vi "OwnMergePanelInventory.vi"() -> ()   [LabVIEW 2024]
panel:
  out "error out":errorcluster caption="错误输出"
  out "pane_ids":refnum<vi>[](array[refnum])
  out "decoration_ids":refnum<vi>[](array[refnum])
  out "all_object_ids":refnum<vi>[](array[refnum])
  in  "target_path":path
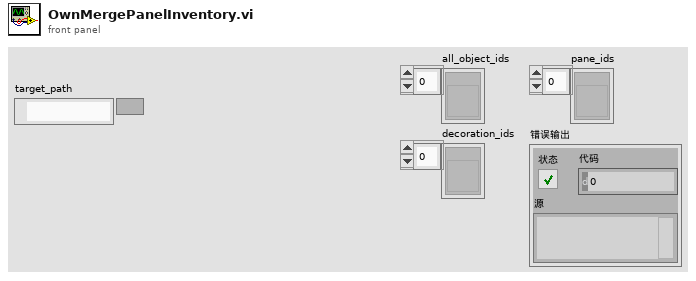
[diagram p1: front panel]
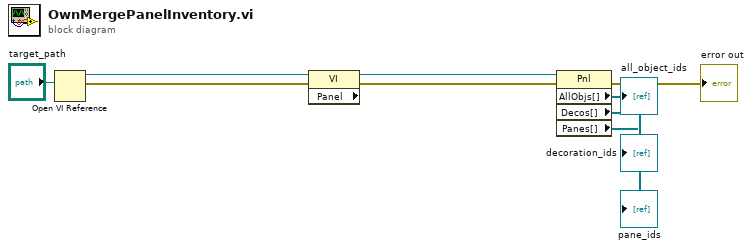
[diagram p0: block diagram]
diagram:
  n1 = Open VI Reference ("打开VI引用")(vi path="target_path") -> (vi reference=w8:refnum<vi>, error out=w7:errorcluster)  [unwired: 5 in]
  n2 = property on="属性节点" class="VI"(reference=w8, error in=w7) -> (error out=w5:errorcluster, "Panel"=w6:refnum<vi>)  [unwired: 1 out]
  n3 = property on="属性节点" class="Pnl"(reference=w6, error in=w5) -> (error out=→"error out":errorcluster, "AllObjs[]"=→"all_object_ids":refnum<vi>[], "Decos[]"=→"decoration_ids":refnum<vi>[], "Panes[]"=→"pane_ids":refnum<vi>[])  [unwired: 1 out]
